vi "Check data length for publish.vi"(9 "Length in":i32=-1, 10 "Offset in":u32, 11 "Data In":u8[](array[numeric])) -> (1 "Length out":u32, 2 "Offset out":u32, 3 "Data out":u8[](array[numeric]))   [LabVIEW 2021, in "Iceoryx.lvlib"]
doc: "If length is -1, use array length\n\nProtect against writing data outside of Data In location:\nCheck that data length is not less than offset, if less set length to 0\nCalculate remaining data and set length to smaller of specified length or remaining data\n\nCould set error if data is limited"
uses:
  Iceoryx.lvlib
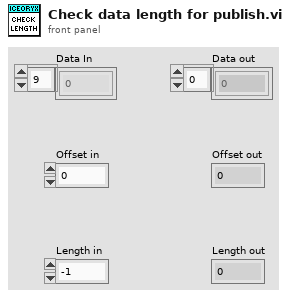
[diagram p1: front panel]
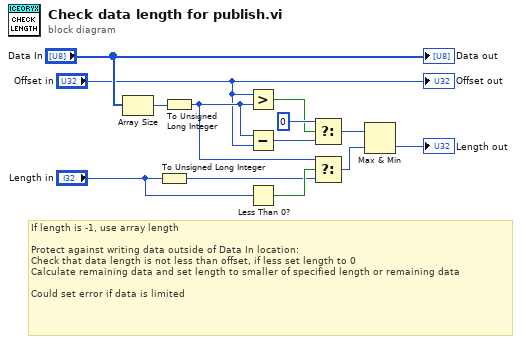
[diagram p0: block diagram]
diagram:
  # "If length is -1, use array length\n\nProtect against writing data outside of Data In location:\nCheck that data length is not less than offset, if less set length to 0\nCalculate remaining data and set length to smaller of specified length or remaining data\n\nCould set error if data is limited"
  n1 = Array Size(array="Data In") -> (size(s)=w9:i32)
  n2 = To Unsigned Long Integer(number="Length in") -> (unsigned 32bit integer=w4:u32)
  n3 = To Unsigned Long Integer(number=w9) -> (unsigned 32bit integer=w6:u32)
  n4 = Greater?(x="Offset in", y=w6) -> (0:w10:bool)
  n5 = Subtract(x=w6, y="Offset in") -> (x-y=w12:u32)
  n6 = Less Than 0?(x="Length in") -> (x < 0?=w7:bool)
  n7 = Select(t=u32 0 ("f"), s=w10, f=w12) -> (s? t:f=w13:u32)
  n8 = Select(t=w6, s=w7, f=w4) -> (s? t:f=w3:u32)
  n9 = Max & Min(x=w13, y=w3) -> (min(x,y)=→"Length out":u32)  [unwired: 1 out]
  "Offset out" <- "Offset in"
  "Data out" <- "Data In"
